vi "set LTE Starting and Num RB.vi"(8 "error in (no error)":errorcluster, 10 "RB Setting Param":T1, 11 "Anritsu Call Box_Implement in":refnum<class "Anritsu Call Box_Implement.lvclass">) -> (0 "error out":errorcluster, 3 "Anritsu Call Box_Implement out":refnum<class "Anritsu Call Box_Implement.lvclass">)   [LabVIEW 2023, in "ANRITSU Call Box.lvlib" / "Anritsu Call Box_Implement.lvclass"]
uses:
  Anritsu Call Box_Implement.lvclass
  Anritsu Call Box_Implement.lvclass/Anritsu Call Box_Implement.ctl
  LTE/LTE.lvclass
  Type Definition/LTE RB Setting Params.ctl
  ANRITSU Call Box.lvlib
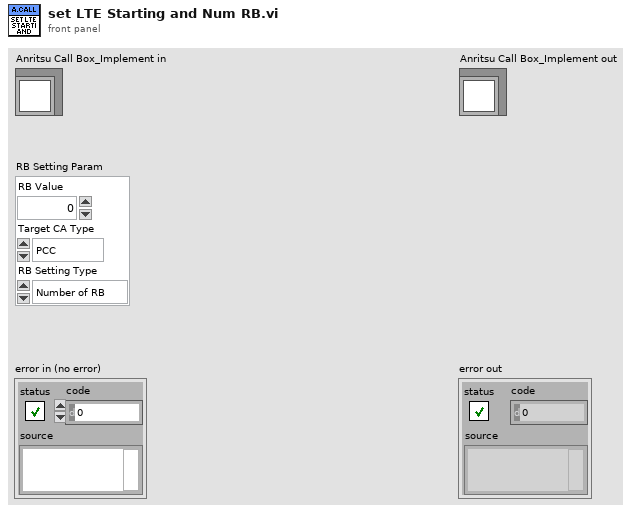
[diagram p1: front panel]
types:
  T1 = typedef "ANRITSU Call Box.lvlib/LTE RB Setting Params.ctl" = cluster{"RB Value":i32, "Target CA Type":enum16{"PCC", "SCC1"}, "RB Setting Type":enum16{"Number of RB", "Starting RB"}}
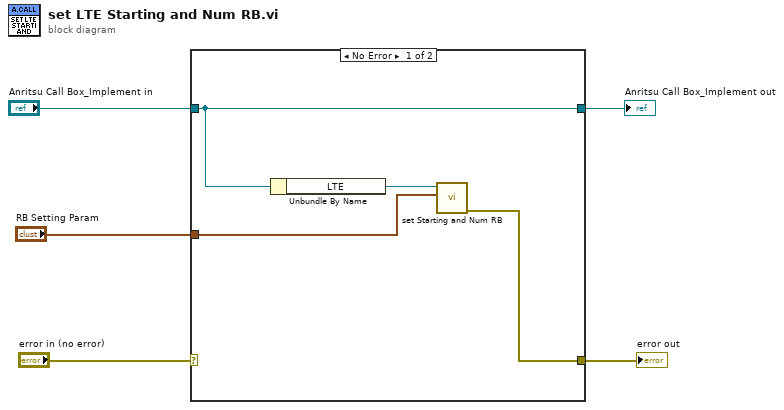
[diagram p0: block diagram]
diagram:
  n1 = case shown="No Error" "error in (no error)" {
    selector: "error in (no error)" -> [_ w10]
    tunnel: "Anritsu Call Box_Implement in" -> [w9 w11]
    tunnel: [w9 w11] -> w4
    tunnel: [w7 w10] -> w2
    tunnel: "RB Setting Param" -> [w6 _]
    frame No Error {
      n2 = Unbundle By Name(w9) -> ("LTE"=w8:refnum<class "LTE.lvclass">)
      n3 = call "set Starting and Num RB.vi"("RB Setting Param"=w6, "LTE in"=w8) -> ("error out"=w7:errorcluster)  [unwired: 8 in, 1 out]
    }
    frame Error {
    }
  }
  "error out" <- w2
  "Anritsu Call Box_Implement out" <- w4
